vi "Measurement Logic.vi"(8 "error in":errorcluster, 9 "measurement configuration":T2={"Automation Test"=FALSE, "Power sequencing file path"="", "RFSG name"="5842_0", "RFSG port"="", "RFSG attenuation mode"=enum."Constant Attenuation", "RFSG external attenuation (dB)"=2.0, "RFSG s-parameters orientation"=enum."Port2 Towards DUT", "RFSG s2p file path"="", "RFmx name"="5842_0", "RFmx port"="", "RFmx attenuation mode"=enum."Constant Attenuation", "RFmx external attenuation (dB)"=1.2, "RFmx s-parameters orientation"=enum."Port2 Towards DUT", "RFmx s2p file path"="", "RFmx Reference Level (dBm)"=10.0, "RFSG Generation IQ Rate (S/s)"=1250000000.0, "Target Pout Per Tone (dBm)"=10.0, "Start Pin Per Tone (dBm)"=10.0, "Start Center Frequency (Hz)"=10.0, "Start Tone Spacing (Hz)"=10.0, "IM_Sweep Mode"=enum."Power", "Sweep Delay (ms)"=10, "Power Sweep End"=10.0, "Power Sweep Step"=10.0, "Frequency Sweep End"=-4.0, "Frequency Sweep Step"=1.0, "Tone Spacing Sweep End"=-4.0, "Tone Spacing Sweep Step"=1.0, "Power sequencing file validity check"=FALSE} {"Tone Spacing Sweep Step" format="%#.pHz"; "Tone Spacing Sweep End" format="%#.pHz"; "Frequency Sweep Step" format="%#.pHz"; "Frequency Sweep End" format="%#.pHz"; "Power Sweep End" format="%#.6f"; "Sweep Delay (ms)" format="%#_6p"; "Start Tone Spacing (Hz)" format="%#.6p"; "Start Center Frequency (Hz)" format="%#.6p"; "Start Pin Per Tone (dBm)" format="%#.6p"; "Target Pout Per Tone (dBm)" format="%#.6f"; "RFSG Generation IQ Rate (S/s)" format="%#.6f"; "RFmx Reference Level (dBm)" format="%#_6p"; "RFmx external attenuation (dB)" format="%.2f"; "RFSG external attenuation (dB)" format="%.2f"}, 10 "measure call context in":refnum<class "Measure Call Context.lvclass">) -> (0 "error out":errorcluster, 1 "measurement results":T1, 2 "measure call context out":refnum<class "Measure Call Context.lvclass">)   [LabVIEW 2023, in "FPT Intermodulation.lvclass"]
doc: "Contains the core logic for executing the measurement."
uses:
  FPT Intermodulation.lvclass
  <vilib>/Plug-In SDKs/Measurements/Measure Call Context/Measure Call Context.lvclass
  Measurement Configuration.ctl
  Measurement Results.ctl
  <extravilib>/ChannelInstances/Event Messenger-bool/Instantiate.vi
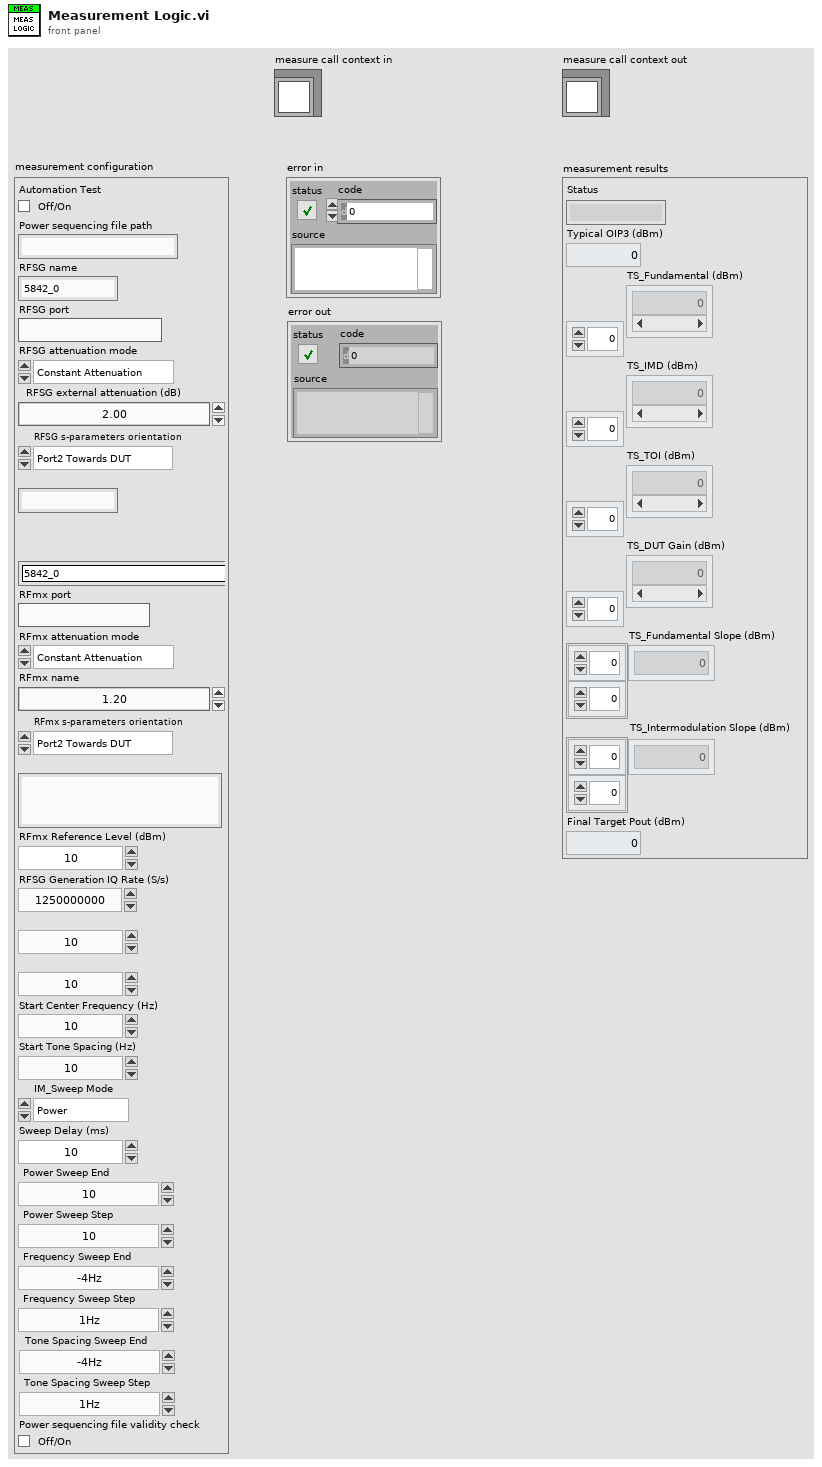
[diagram p1: front panel]
types:
  T1 = typedef "FPT Intermodulation.lvclass/Measurement Results.ctl" = cluster{"Status":string, "Typical OIP3 (dBm)":dbl, "TS_Fundamental (dBm)":dbl[][], "TS_IMD (dBm)":dbl[][], "TS_TOI (dBm)":dbl[][], "TS_DUT Gain (dBm)":dbl[][], "TS_Fundamental Slope (dBm)":dbl[][], "TS_Intermodulation Slope (dBm)":dbl[][], "Final Target Pout (dBm)":dbl}
  T2 = typedef "FPT Intermodulation.lvclass/Measurement Configuration.ctl" = cluster{"Automation Test":bool, "Power sequencing file path":string, "RFSG name":string, "RFSG port":string, "RFSG attenuation mode":enum32{"<None>", "Constant Attenuation", "s2p File"}, "RFSG external attenuation (dB)":dbl, "RFSG s-parameters orientation":enum32{"Port1 Towards DUT", "Port2 Towards DUT"}, "RFSG s2p file path":string, "RFmx name":string, "RFmx port":string, "RFmx attenuation mode":enum32{"<None>", "Constant Attenuation", "s2p File"}, "RFmx external attenuation (dB)":dbl, "RFmx s-parameters orientation":enum32{"Port1 Towards DUT", "Port2 Towards DUT"}, "RFmx s2p file path":string, "RFmx Reference Level (dBm)":dbl, "RFSG Generation IQ Rate (S/s)":dbl, "Target Pout Per Tone (dBm)":dbl, "Start Pin Per Tone (dBm)":dbl, "Start Center Frequency (Hz)":dbl, "Start Tone Spacing (Hz)":dbl, "IM_Sweep Mode":enum32{"Power", "Frequency", "Tone Spacing"}, "Sweep Delay (ms)":u32, "Power Sweep End":dbl, "Power Sweep Step":dbl, "Frequency Sweep End":dbl, "Frequency Sweep Step":dbl, "Tone Spacing Sweep End":dbl, "Tone Spacing Sweep Step":dbl, "Power sequencing file validity check":bool}
  T3 = enum32{"Power On Dut", "De-embedding + Measurement", "Power Off Dut"}[]
  T4 = cluster{"measurement configuration":T2, "measurement results":T1, "CustomData":cluster{"Valid CSV":bool}}
  T5 = typedef "RFmx Config - TOI.ctl" = cluster{"Reference Level (dBm)":dbl, "Attenuation":T6}
  T6 = typedef "RFmx Config.ctl" = cluster{"RFmx Name":refnum<k15>, "RFmx Port":string, "Attenuation":cluster{"Mode":enum32{"<None>", "Constant Attenuation", "s2p File"}, "Constant Attenuation":cluster{"RFmx External Attenuation (dB)":dbl}, "s2p File":cluster{"RFmx S-Parameters Orientation":i32, "RFmx Attenuation s2p Path Name":string, "RFmx Attenuation s2p File":path}}}
  T7 = typedef "RFSG Config - TOI.ctl" = cluster{"IQ Rate (S/sec)":dbl, "Number of Samples":i32, "Attenuation":T8}
  T8 = typedef "RFsg Config.ctl" = cluster{"RFSG Name":refnum<k15>, "RFSG Port":string, "Attenuation":cluster{"Mode":enum32{"<None>", "Constant Attenuation", "s2p File"}, "Contant Attenuation":cluster{"RFSG External Attenuation (dB)":dbl}, "s2p File":cluster{"RFSG S-parameters Orientation":i32, "RFSG Attenuation s2p Path Name":string, "RFSG s2p File Path":path}}}
  T9 = typedef "Test Config - TOI.ctl" = cluster{"Target Pout Per Tone (dBm)":dbl, "Start Value":cluster{"Power Level per Tone (dBm)":dbl, "Center Frequency (Hz)":dbl, "Tone Spacing (Hz)":dbl}, "Sweep Settings":cluster{"Mode":enum16{"Power", "Frequency", "Tone Spacing"}, "Sweep Delay (ms)":u32, "Power Sweep End":dbl, "Power Sweep Step":dbl, "Frequency Sweep End":dbl, "Frequency Sweep Step":dbl, "Tone Spacing Sweep End":dbl, "Tone Spacing Sweep Step":dbl}}
  T10 = typedef "Target Pout per Tone Results Cluster - TOI.ctl" = cluster{"Target Pout per Tone (dBm)":dbl, "OIP3 (dBm)":dbl, "IIP3 (dBm)":dbl, "Pin per Tone (dBm)":dbl, "IMD (dBm)":dbl}
  T11 = typedef "Event Messenger-bool.lvlib/))Channel.ctl" = refnum<queue>
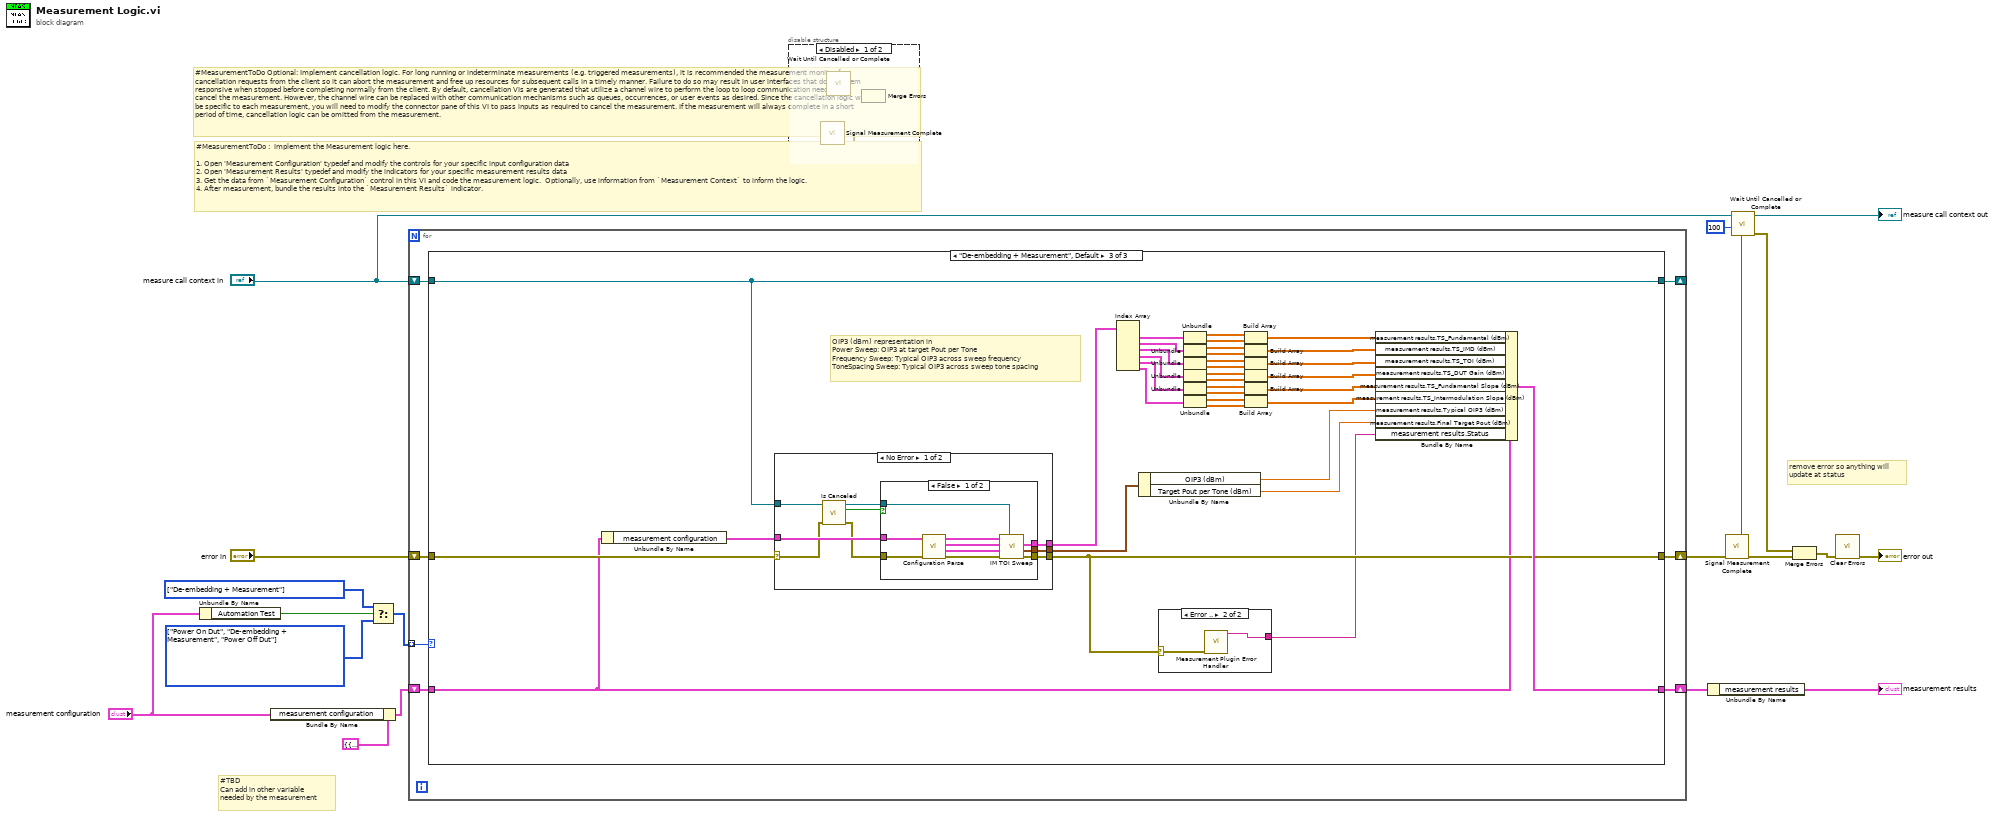
[diagram p0: block diagram]
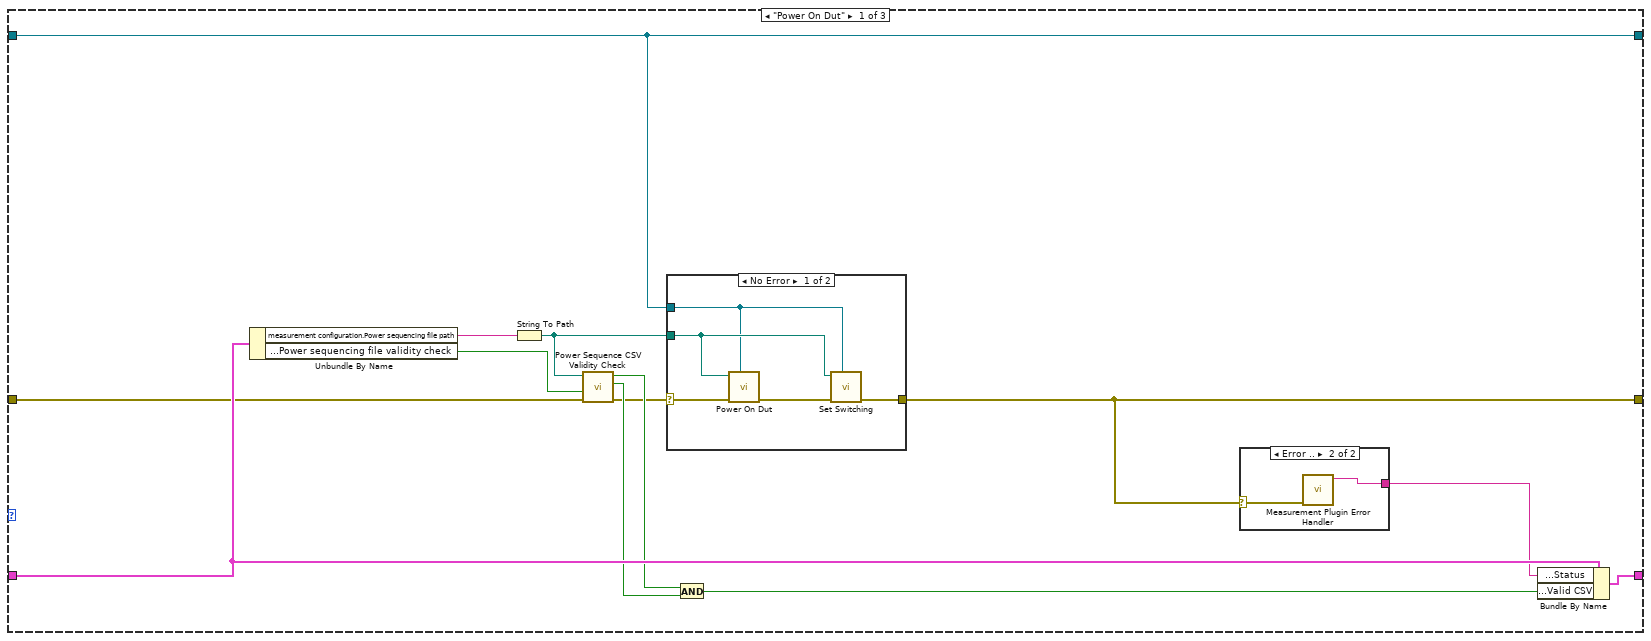
[diagram p2: hidden frame]
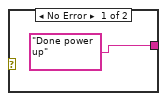
[diagram p4: hidden frame]
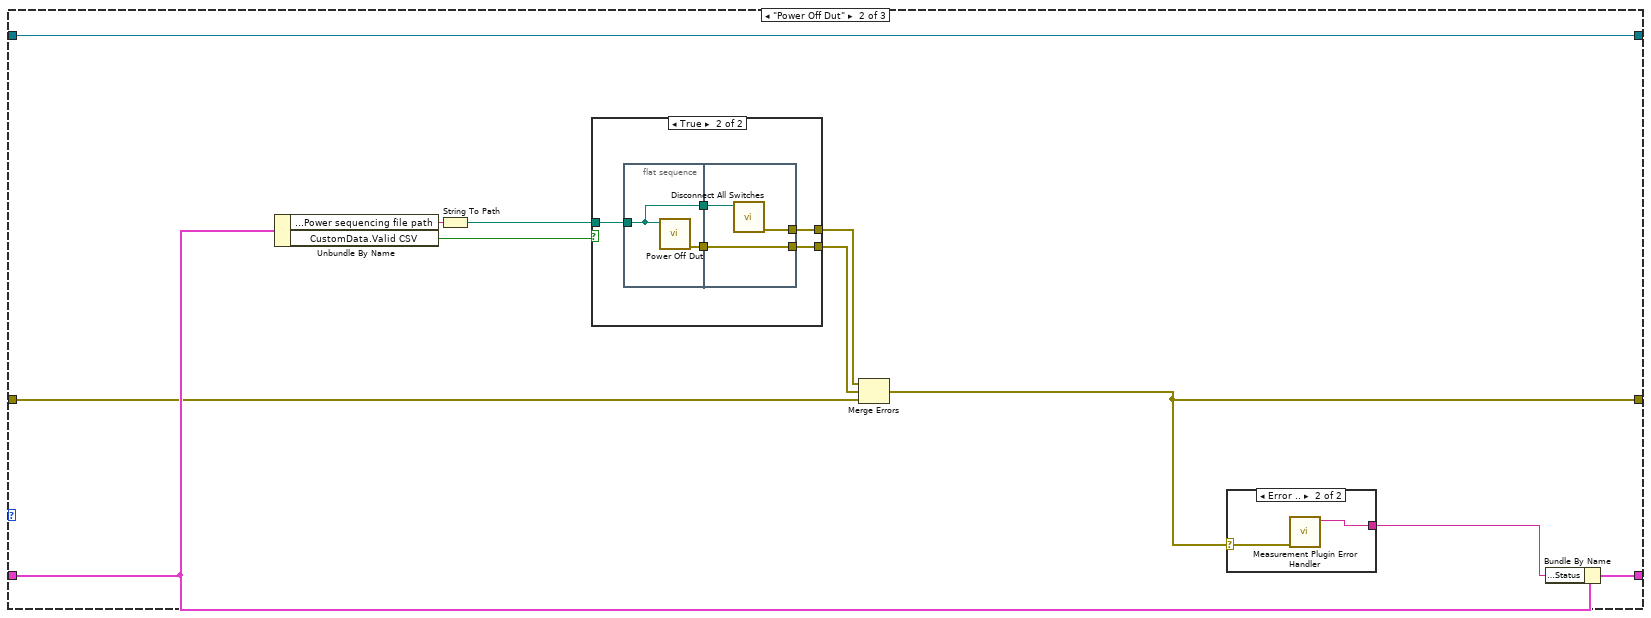
[diagram p5: hidden frame]
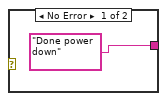
[diagram p7: hidden frame]
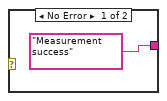
[diagram p8: hidden frame]
diagram:
  w9 = T3 [enum."De-embedding + Measurement"] items=["Power On Dut", "De-embedding + Measurement", "Power Off Dut"]
  w13 = T3 [enum."Power On Dut", enum."De-embedding + Measurement", enum."Power Off Dut"] items=["Power On Dut", "De-embedding + Measurement", "Power Off Dut"]
  # "remove error so anything will\nupdate at status"
  # "#TBD\nCan add in other variable\nneeded by the measurement"
  # "#MeasurementToDo Optional: Implement cancellation logic. For long running or indeterminate measurements (e.g. triggered measurements), it is recommended the measurement monitor for cancellation requests from the client so it can abort the measurement and free up resources for subsequent calls in a timely manner. Failure to do so may result in user interfaces that do not seem responsive when stopped before completing normally from the client. By default, cancellation VIs are generated that utilize a channel wire to perform the loop to loop communication needed to cancel the measurement. However, the channel wire can be replaced with other communication mechanisms such as queues, occurrences, or user events as desired. Since the cancellation logic will be specific to each measurement, you will need to modify the connector pane of this VI to pass inputs as required to cancel the measurement. If the measurement will always complete in a short period of time, cancellation logic can be omitted from the measurement."
  # "#MeasurementToDo :  Implement the Measurement logic here.\n\n1. Open 'Measurement Configuration' typedef and modify the controls for your specific input configuration data\n2. Open 'Measurement Results' typedef and modify the indicators for your specific measurement results data\n3. Get the data from `Measurement Configuration` control in this VI and code the measurement logic.  Optionally, use information from `Measurement Context` to inform the logic.\n4. After measurement, bundle the results into the `Measurement Results` indicator."
  n1 = Unbundle By Name("measurement configuration") -> ("Automation Test"=w10:bool)
  n2 = Bundle By Name(cluster=T4 {"measurement configuration"={"Automation Test"=FALSE, "Power sequencing file path"="", "RFSG name"="5842_0", "RFSG port"="", "RFSG attenuation mode"=enum."Constant Attenuation", "RFSG external attenuation (dB)"=2.0, "RFSG s-parameters orientation"=enum."Port2 Towards DUT", "RFSG s2p file path"="", "RFmx name"="5842_0", "RFmx port"="", "RFmx attenuation mode"=enum."Constant Attenuation", "RFmx external attenuation (dB)"=1.2, "RFmx s-parameters orientation"=enum."Port2 Towards DUT", "RFmx s2p file path"="", "RFmx Reference Level (dBm)"=10.0, "RFSG Generation IQ Rate (S/s)"=1250000000.0, "Target Pout Per Tone (dBm)"=10.0, "Start Pin Per Tone (dBm)"=10.0, "Start Center Frequency (Hz)"=10.0, "Start Tone Spacing (Hz)"=10.0, "IM_Sweep Mode"=enum."Power", "Sweep Delay (ms)"=10, "Power Sweep End"=10.0, "Power Sweep Step"=10.0, "Frequency Sweep End"=-4.0, "Frequency Sweep Step"=1.0, "Tone Spacing Sweep End"=-4.0, "Tone Spacing Sweep Step"=1.0, "Power sequencing file validity check"=FALSE}, "measurement results"={"Status"="", "Typical OIP3 (dBm)"=0.0, "TS_Fundamental (dBm)"=[], "TS_IMD (dBm)"=[], "TS_TOI (dBm)"=[], "TS_DUT Gain (dBm)"=[], "TS_Fundamental Slope (dBm)"=[], "TS_Intermodulation Slope (dBm)"=[], "Final Target Pout (dBm)"=0.0}, "CustomData"={"Valid CSV"=FALSE}}, "measurement configuration"="measurement configuration") -> (w17:T4)
  n3 = Select(t=w9, s=w10, f=w13) -> (s? t:f=w12:T3)
  n4 = for {
    tunnel: w12 -> [w25] mode=indexing
    shift-right: [w20] -> w8
    shift-left: "error in" -> [w26]
    shift-right: [w21] -> w16
    shift-left: w17 -> [w24]
    shift-right: [w22] -> _
    shift-left: "measure call context in" -> [w23]
    n5 = case shown="\"De-embedding + Measurement\", Default" w25 {
      tunnel: w26 -> [w28 w54 w86]
      tunnel: w24 -> [w39 w55 w85]
      tunnel: w23 -> [w34 w58 w74]
      tunnel: [w35 w53 w106] -> w20
      tunnel: [w34 w58 w74] -> w22
      tunnel: [w37 w56 w107] -> w21
      frame "Power On Dut" {
        n6 = Unbundle By Name(w39) -> ("measurement configuration.Power sequencing file path"=w36:string, "measurement configuration.Power sequencing file validity check"=w29:bool)
        n7 = String To Path(string=w36) -> (path=w33:path)
        n8 = call "Power Sequence CSV Validity Check.vi"("error in"=w28, "Enable Validity Check?"=w29, "File Path"=w33) -> ("error out"=w27:errorcluster, "Valid Execution Order"=w32:bool, "All Instruments Available"=w31:bool)  [unwired: 5 in, 1 out]
        n9 = case shown="No Error" w27 {
          selector: w27 -> [w40 w45]
          tunnel: [w43 w45] -> w35
          tunnel: w33 -> [w42 _]
          tunnel: w34 -> [w41 _]
          frame No Error {
            n10 = call "Power On Dut.vi"("measure call context in"=w41, "error in"=w40, "Power sequencing file path"=w42) -> ("error out"=w44:errorcluster)  [unwired: 7 in, 1 out]
            n11 = call "Set Switching.vi"("measure call context in"=w41, "error in"=w44, "File Path"=w42) -> ("error out"=w43:errorcluster)  [unwired: 7 in, 1 out]
          }
          frame Error {
          }
        }
        n12 = And(x=w31, y=w32) -> (x .and. y?=w30:bool)
        n13 = case shown="Error .." w35 {
          selector: w35 -> [_ w48]
          tunnel: ["Done power up" w47] -> w38
          frame No Error {
          }
          frame Error {
            n14 = call "Measurement Plugin Error Handler.vi"("error in"=w48) -> ("Status Message (Error)"=w47:string)  [unwired: 9 in, 1 out]
          }
        }
        n15 = Bundle By Name(cluster=w39, "measurement results.Status"=w38, "CustomData.Valid CSV"=w30) -> (w37:T4)
      }
      frame "Power Off Dut" {
        n16 = Unbundle By Name(w55) -> ("measurement configuration.Power sequencing file path"=w59:string, "CustomData.Valid CSV"=w49:bool)
        n17 = String To Path(string=w59) -> (path=w52:path)
        n18 = case shown="True" w49 {
          tunnel: w52 -> [_ w62]
          tunnel: [_ w61] -> w51
          tunnel: [_ w60] -> w50
          frame False {
          }
          frame True {
            n19 = flat-sequence {
              tunnel: w62 -> [w65]
              tunnel: [w66] -> w64
              tunnel: [w65] -> w63
              tunnel: [w69] -> w60
              tunnel: w64 -> [w69]
              tunnel: [w68] -> w61
              tunnel: w63 -> [w67]
              frame #0 {
                n20 = call "Power Off Dut.vi"("Power Sequencing File Path"=w65) -> ("error out"=w66:errorcluster)  [unwired: 10 in]
              }
              frame #1 {
                n21 = call "Disconnect All Switches.vi"("File Path"=w67) -> ("error out"=w68:errorcluster)  [unwired: 10 in]
              }
            }
          }
        }
        n22 = Merge Errors(w51, w50, w54) -> (w53:errorcluster)
        n23 = case shown="Error .." w53 {
          selector: w53 -> [_ w72]
          tunnel: ["Done power down" w71] -> w57
          frame No Error {
          }
          frame Error {
            n24 = call "Measurement Plugin Error Handler.vi"("error in"=w72) -> ("Status Message (Error)"=w71:string)  [unwired: 9 in, 1 out]
          }
        }
        n25 = Bundle By Name(cluster=w55, "measurement results.Status"=w57) -> (w56:T4)
      }
      frame "De-embedding + Measurement", Default {
        # "OIP3 (dBm) representation in\nPower Sweep: OIP3 at target Pout per Tone\nFrequency Sweep: Typical OIP3 across sweep frequency\nToneSpacing Sweep: Typical OIP3 across sweep tone spacing"
        n26 = Unbundle By Name(w85) -> ("measurement configuration"=w73:T2)
        n27 = case shown="No Error" w86 {
          selector: w86 -> [w113 w131]
          tunnel: [w119 w131] -> w106
          tunnel: [w118 _] -> w105
          tunnel: [w117 _] -> w100
          tunnel: w73 -> [w116 _]
          tunnel: w74 -> [w112 _]
          frame No Error {
            n28 = call <vilib>:"Is Canceled.vi"("error in"=w113, "measure call context in"=w112) -> ("error out"=w114:errorcluster, "is canceled?"=w115:bool, "measure call context out"=w111:refnum<class "Measure Call Context.lvclass">)  [unwired: 7 in]
            n29 = case shown="False" w115 {
              tunnel: [w129 w130] -> w119
              tunnel: [w128 _] -> w118
              tunnel: [w127 _] -> w117
              tunnel: w116 -> [w122 _]
              tunnel: w114 -> [w121 w130]
              tunnel: w111 -> [w120 _]
              frame False {
                n30 = call "Configuration Parse.vi"("error in"=w121, "Measurement Configuration"=w122) -> ("error out"=w126:errorcluster, "RFmx Settings"=w123:T5, "RFSG Settings"=w124:T7, "Test Configuration"=w125:T9)  [unwired: 6 in]
                n31 = call "IM TOI Sweep.vi"("measure call context in"=w120, "error in"=w126, "RFmx Settings"=w123, "RFSG Settings"=w124, "Test Configuration"=w125) -> ("error out"=w129:errorcluster, "Power Sweep Results - Target Pout per Tone"=w127:T10, "TOI Plot"=w128:cluster{dbl[], dbl[]}[])  [unwired: 2 in, 2 out]
              }
              frame True {
              }
            }
          }
          frame Error {
          }
        }
        n32 = Index Array(array=w105) -> (element #1=w104:cluster{dbl[], dbl[]}, element #2=w103:cluster{dbl[], dbl[]}, element #3=w102:cluster{dbl[], dbl[]}, element #4=w101:cluster{dbl[], dbl[]}, element #5=w78:cluster{dbl[], dbl[]}, element #6=w77:cluster{dbl[], dbl[]})  [unwired: 6 in]
        n33 = Unbundle By Name(w100) -> ("OIP3 (dBm)"=w87:dbl, "Target Pout per Tone (dBm)"=w83:dbl)
        n34 = case shown="Error .." w106 {
          selector: w106 -> [_ w110]
          tunnel: ["Measurement success" w109] -> w84
          frame No Error {
          }
          frame Error {
            n35 = call "Measurement Plugin Error Handler.vi"("error in"=w110) -> ("Status Message (Error)"=w109:string)  [unwired: 9 in, 1 out]
          }
        }
        n36 = Unbundle(w104) -> (w99:dbl[], w98:dbl[])
        n37 = Unbundle(w103) -> (w96:dbl[], w95:dbl[])
        n38 = Unbundle(w102) -> (w93:dbl[], w92:dbl[])
        n39 = Unbundle(w101) -> (w89:dbl[], w90:dbl[])
        n40 = Unbundle(w78) -> (w82:dbl[], w81:dbl[])
        n41 = Unbundle(w77) -> (w80:dbl[], w79:dbl[])
        n42 = Build Array(w99, w98) -> (w97:dbl[][])
        n43 = Build Array(w96, w95) -> (w94:dbl[][])
        n44 = Build Array(w93, w92) -> (w91:dbl[][])
        n45 = Build Array(w89, w90) -> (w88:dbl[][])
        n46 = Build Array(w82, w81) -> (w76:dbl[][])
        n47 = Build Array(w80, w79) -> (w75:dbl[][])
        n48 = Bundle By Name(cluster=w85, "measurement results.TS_Fundamental (dBm)"=w97, "measurement results.TS_IMD (dBm)"=w94, "measurement results.TS_TOI (dBm)"=w91, "measurement results.TS_DUT Gain (dBm)"=w88, "measurement results.TS_Fundamental Slope (dBm)"=w76, "measurement results.TS_Intermodulation Slope (dBm)"=w75, "measurement results.Typical OIP3 (dBm)"=w87, "measurement results.Final Target Pout (dBm)"=w83, "measurement results.Status"=w84) -> (w107:T4)
      }
    }
  }
  n49 = disable-structure shown="Disabled" {
    frame Disabled {
      n50 = call "Signal Measurement Complete.vi"() -> ("error out"=w133:errorcluster, "done channel"=w134:T11)  [unwired: 10 in]
      n51 = call "Wait Until Cancelled or Complete.vi"("done channel"=w134) -> ("error out"=w132:errorcluster)  [unwired: 9 in, 1 out]
      n52 = Merge Errors(w132, w133) -> ()  [unwired: 1 out]
    }
    frame Enabled {
    }
  }
  n53 = Unbundle By Name(w16) -> ("measurement results"=→"measurement results":T1)
  n54 = call "Signal Measurement Complete.vi"("error in (no error)"=w8) -> ("error out"=w7:errorcluster, "done channel"=w5:T11)  [unwired: 9 in]
  n55 = call "Wait Until Cancelled or Complete.vi"("done channel"=w5, "ms polling interval"=100, "measure call context in"="measure call context in") -> ("error out"=w3:errorcluster, "measure call context out"=→"measure call context out":refnum<class "Measure Call Context.lvclass">)  [unwired: 7 in]
  n56 = Merge Errors(w3, w7) -> (w4:errorcluster)
  n57 = call <vilib>:"Clear Errors.vi"("error in (no error)"=w4) -> ("error out"=→"error out":errorcluster)  [unwired: 5 in, 1 out]
